vi "数据保存判断.vi"(11 "appended path":path) -> (3 "数据保存中?":bool)   [LabVIEW 2026, in "UI-无创.lvlib"]
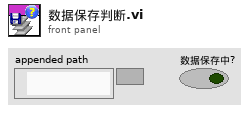
[diagram p1: front panel]
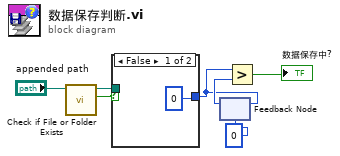
[diagram p0: block diagram]
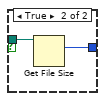
[diagram p2: hidden frame]
diagram:
  n1 = call <vilib>:"Check if File or Folder Exists.vi"("path"="appended path") -> ("file or folder exists?"=w2:bool, "dup path"=w1:path)  [unwired: 8 in, 1 out]
  n2 = case shown="False" w2 {
    tunnel: w1 -> [_ w10]
    tunnel: [i64 0 ("大小（字节）") w9] -> w3
    frame False {
    }
    frame True {
      n3 = Get File Size(file=w10) -> (size (in bytes)=w9:i64)  [unwired: 1 in, 2 out]
    }
  }
  n4 = feedback #1(i64 0) -> (w4:i64)
  n5 = feedback-in #1(w3) -> ()
  n6 = Greater?(x=w3, y=w4) -> (0:→"数据保存中?":bool)
